vi "ZM-HW-SIM-randomData.vi"(8 "error in (no error)":errorcluster) -> (0 "error out":errorcluster, 3 "data":T1)   [LabVIEW 2020, in "ZM-HW-SIM-simulated_hardware.lvlib" / "ZM-HW-SIM-simulated_hardware.lvclass"]
doc: "Random test data for the simulated hardware: temperature_c in [20, 30), sample_index 0-999, duty_percent 0-100, sensor_ok mostly TRUE, status ok, warm or cold, as a ZM-PC-TP-DATA cluster. No node here raises an error."
uses:
  ZM-HW-SIM-simulated_hardware.lvclass
  common/ZM-PC-packages/ZM-PC-TP-test_package/ZM-PC-TP-DATA.ctl
  common/ZM-PC-packages/ZM-PC-TP-test_package/ZM-PC-TP-test_package.lvclass
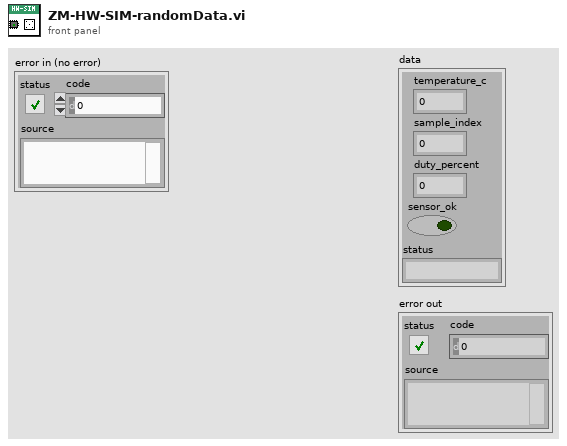
[diagram p1: front panel]
types:
  T1 = typedef "ZM-PC-packages.lvlib/ZM-PC-TP-test_package.lvclass/ZM-PC-TP-DATA.ctl" = cluster{"temperature_c":dbl, "sample_index":i32, "duty_percent":u8, "sensor_ok":bool, "status":string}
  T2 = cluster{"temperature_c":dbl, "sample_index":i32, "duty_percent":u8, "sensor_ok":bool, "status":string}
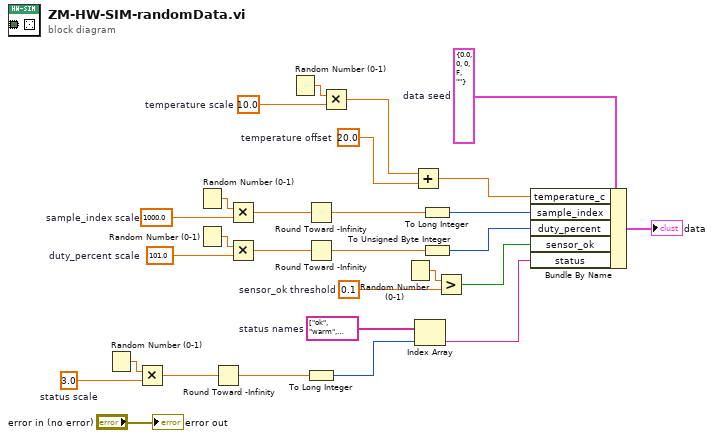
[diagram p0: block diagram]
diagram:
  w3 = T2 {"temperature_c"=0.0, "sample_index"=0, "duty_percent"=0, "sensor_ok"=FALSE, "status"=""}  # data seed
  w10 = string[] ["ok", "warm", "cold"]  # status names
  w13 = 3.0  # status scale
  w15 = 0.1  # sensor_ok threshold
  w19 = 101.0  # duty_percent scale
  w23 = 1000.0  # sample_index scale
  w25 = 20.0  # temperature offset
  w27 = 10.0  # temperature scale
  n1 = Random Number (0-1)() -> (number: 0 to 1=w14:dbl)
  n2 = Multiply(x=w14, y=w13) -> (x*y=w12:dbl)
  n3 = Random Number (0-1)() -> (number: 0 to 1=w24:dbl)
  n4 = Random Number (0-1)() -> (number: 0 to 1=w20:dbl)
  n5 = Round Toward -Infinity(1:w12) -> (0:w11:dbl)
  n6 = Multiply(x=w24, y=w23) -> (x*y=w22:dbl)
  n7 = Multiply(x=w20, y=w19) -> (x*y=w18:dbl)
  n8 = Random Number (0-1)() -> (number: 0 to 1=w28:dbl)
  n9 = Round Toward -Infinity(1:w22) -> (0:w21:dbl)
  n10 = Round Toward -Infinity(1:w18) -> (0:w17:dbl)
  n11 = To Long Integer(number=w11) -> (32bit integer=w9:i32)
  n12 = Multiply(x=w28, y=w27) -> (x*y=w26:dbl)
  n13 = Random Number (0-1)() -> (number: 0 to 1=w16:dbl)
  n14 = Add(x=w26, y=w25) -> (x+y=w8:dbl)
  n15 = Index Array(array=w10, index=w9) -> (element=w4:string)
  n16 = To Long Integer(number=w21) -> (32bit integer=w7:i32)
  n17 = To Unsigned Byte Integer(number=w17) -> (unsigned 8bit integer=w6:u8)
  n18 = Greater?(x=w16, y=w15) -> (0:w5:bool)
  n19 = Bundle By Name(cluster=w3, "temperature_c"=w8, "sample_index"=w7, "duty_percent"=w6, "sensor_ok"=w5, "status"=w4) -> (→"data":T2)
  "error out" <- "error in (no error)"
